vi "Run TS.vi"(8 "error in":errorcluster, 11 "Test Stand in":refnum<class "Generic Test Stand.lvclass">) -> (0 "error out":errorcluster, 3 "Test Stand out":refnum<class "Generic Test Stand.lvclass">)   [LabVIEW 2019, in "Generic Test Stand.lvclass"]
uses:
  Generic Test Stand.lvclass
  Generic Test Stand.lvclass/Generic Test Stand.ctl
  DAC/DAC.lvclass
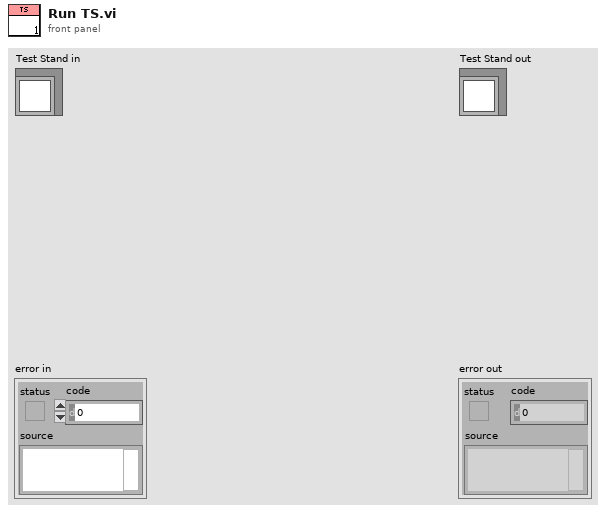
[diagram p1: front panel]
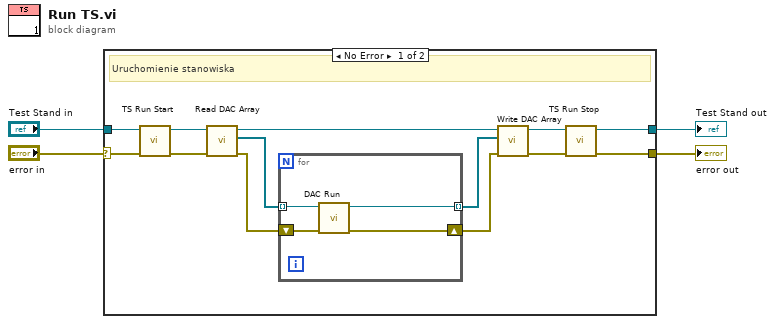
[diagram p0: block diagram]
diagram:
  n1 = case shown="No Error" "error in" {
    selector: "error in" -> [w7 w23]
    tunnel: "Test Stand in" -> [w8 w22]
    tunnel: [w10 w22] -> w3
    tunnel: [w9 w23] -> w1
    frame No Error {
      # "Uruchomienie stanowiska"
      n2 = call-dynamic "TS Run Start.vi"("error in (no error)"=w7, "Test Stand in"=w8) -> ("error out"=w6:errorcluster, "Test Stand out"=w13:refnum<class "Generic Test Stand.lvclass">)  [unwired: 8 in]
      n3 = call "Read DAC Array.vi"("error in (no error)"=w6, "Generic Test Stand in"=w13) -> ("error out"=w5:errorcluster, "DAC Array"=w17:refnum<class "DAC.lvclass">[], "Generic Test Stand out"=w16:refnum<class "Generic Test Stand.lvclass">)  [unwired: 7 in]
      n4 = for {
        tunnel: w17 -> [w21] mode=indexing
        shift-right: [w18] -> w14
        shift-left: w5 -> [w20]
        tunnel: [w19] -> w15 mode=indexing
        n5 = call-dynamic "DAC Run.vi"("error in (no error)"=w20, "DAC in"=w21) -> ("error out"=w18:errorcluster, "DAC out"=w19:refnum<class "DAC.lvclass">)  [unwired: 8 in]
      }
      n6 = call "Write DAC Array.vi"("error in (no error)"=w14, "DAC Array"=w15, "Generic Test Stand in"=w16) -> ("error out"=w11:errorcluster, "Generic Test Stand out"=w12:refnum<class "Generic Test Stand.lvclass">)  [unwired: 7 in]
      n7 = call-dynamic "TS Run Stop.vi"("error in (no error)"=w11, "Test Stand in"=w12) -> ("error out"=w9:errorcluster, "Test Stand out"=w10:refnum<class "Generic Test Stand.lvclass">)  [unwired: 8 in]
    }
    frame Error {
    }
  }
  "error out" <- w1
  "Test Stand out" <- w3
